vi "Parameters_Get_Reference.vi"(8 "error in (no error)":errorcluster, 11 "Parameters":dbl[](array[numeric])) -> (0 "error out":errorcluster, 2 "Reference Move Parameters":T1={"Reference Move Mode"=11599899, "Start Search Forward"=FALSE, "Stop on FWD Edge"=FALSE, "Approach Forward"=FALSE, "Velocity"=0.0, "Acceleration"=0.0} {"Reference Move Mode" items=["Home"=11599899, "Index"=11599900, "Center"=11599901, "Forward Limit"=11599902, "Reverse Limit"=11599903, "Absolute"=12648450]}, 3 "Axis to command":i32)   [LabVIEW 2017, in "WordManipulationLibrary.lvlib"]
uses:
  WordManipulationLibrary.lvlib
  Parameters_Reference.ctl
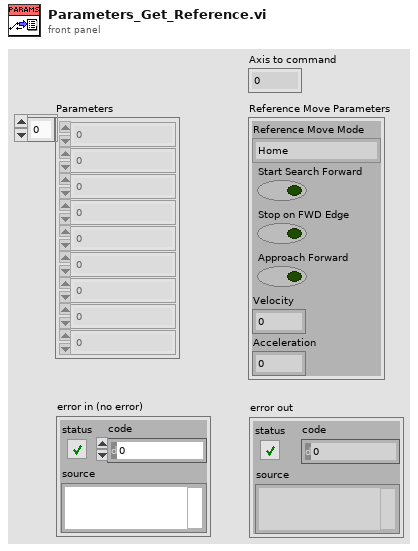
[diagram p1: front panel]
types:
  T1 = typedef "WordManipulationLibrary.lvlib/Parameters_Reference.ctl" = cluster{"Reference Move Mode":i32, "Start Search Forward":bool, "Stop on FWD Edge":bool, "Approach Forward":bool, "Velocity":dbl, "Acceleration":dbl}
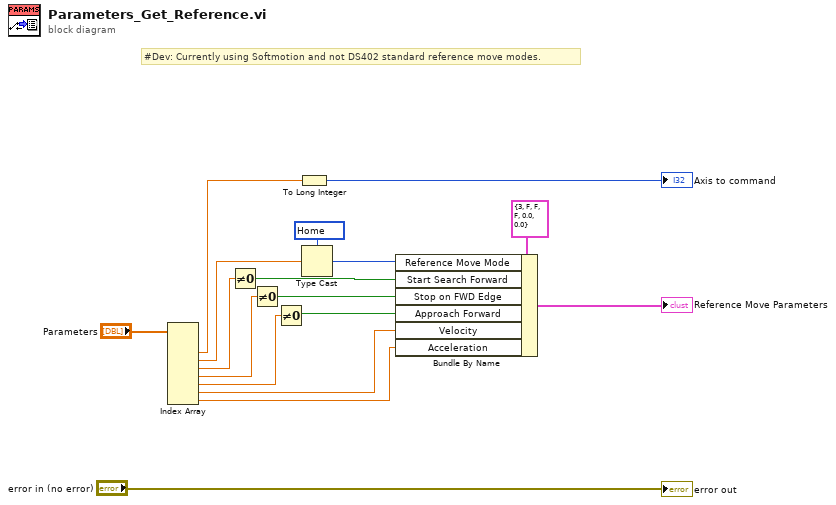
[diagram p0: block diagram]
diagram:
  w1 = 11599899 items=["Home"=11599899, "Index"=11599900, "Center"=11599901, "Forward Limit"=11599902, "Reverse Limit"=11599903, "Absolute"=12648450] ("Reference Move Mode")
  # "#Dev: Currently using Softmotion and not DS402 standard reference move modes."
  n1 = Index Array(array="Parameters") -> (element #2=w5:dbl, element #3=w3:dbl, element #4=w12:dbl, element #5=w11:dbl, element #6=w10:dbl, element #7=w9:dbl, element #8=w13:dbl)  [unwired: 8 in, 1 out]
  n2 = Not Equal To 0?(x=w12) -> (x != 0?=w8:bool)
  n3 = Not Equal To 0?(x=w11) -> (x != 0?=w7:bool)
  n4 = Not Equal To 0?(x=w10) -> (x != 0?=w6:bool)
  n5 = To Long Integer(number=w5) -> (32bit integer=→"Axis to command":i32)
  n6 = Type Cast(type=w1, x=w3) -> (*(type *) &x=w2:i32)
  n7 = Bundle By Name(cluster=T1 {"Reference Move Mode"=3, "Start Search Forward"=FALSE, "Stop on FWD Edge"=FALSE, "Approach Forward"=FALSE, "Velocity"=0.0, "Acceleration"=0.0} ("output cluster 2"), "Reference Move Mode"=w2, "Start Search Forward"=w8, "Stop on FWD Edge"=w7, "Approach Forward"=w6, "Velocity"=w9, "Acceleration"=w13) -> (→"Reference Move Parameters":T1)
  "error out" <- "error in (no error)"
